vi "DSS-Tests-golden_read.vi"(8 "error in":errorcluster, 11 "file path":path) -> (0 "error out":errorcluster, 2 "found":bool, 3 "values":dbl[](array[numeric]))   [LabVIEW 2020, in "DSS-Tests.lvlib"]
doc: "Reads a golden text file of one value per line (period as decimal point) into a 1D DBL array; found is false and the array empty when the file does not exist."
uses:
  DSS-Tests.lvlib
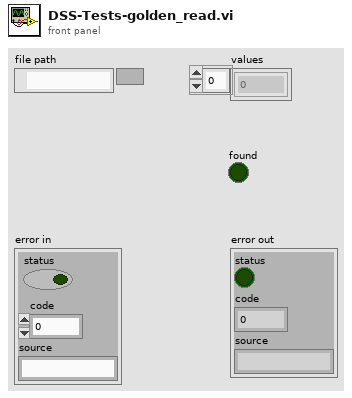
[diagram p1: front panel]
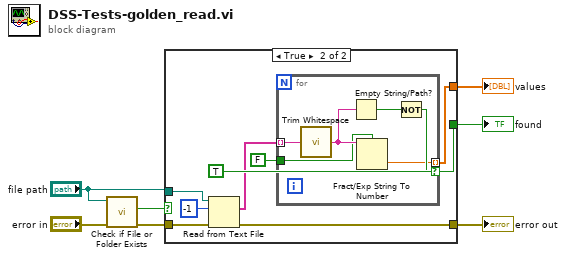
[diagram p0: block diagram]
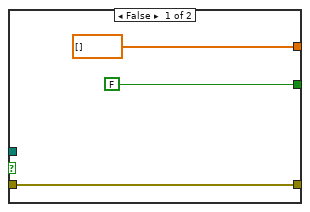
[diagram p2: hidden frame]
diagram:
  n1 = call <vilib>:"Check if File or Folder Exists.vi"("error in (no error)"="error in", "path"="file path") -> ("error out"=w3:errorcluster, "file or folder exists?"=w4:bool)  [unwired: 7 in, 1 out]
  n2 = case shown="True" w4 {
    tunnel: "file path" -> [_ w11]
    tunnel: [FALSE ("not found") TRUE ("found")] -> w6
    tunnel: w3 -> [w8 w12]
    tunnel: [w8 w15] -> w7
    tunnel: [dbl[] [] ("no values") w17] -> w5
    frame False {
    }
    frame True {
      n3 = Read from Text File(file (use dialog)=w11, count=-1, error in=w12) -> (text=w14:string[], error out=w15:errorcluster)  [unwired: 1 in, 2 out]
      n4 = for {
        tunnel: FALSE ("use system decimal point (T)") -> [w20]
        tunnel: w14 -> [w19] mode=indexing
        tunnel: [w22] -> w17 mode=indexing if=w24
        n5 = call <vilib>:"Trim Whitespace.vi"("string"=w19) -> ("trimmed string"=w21:string)  [unwired: 1 in]
        n6 = Empty String/Path?(string/path=w21) -> (empty?=w23:bool)
        n7 = Fract/Exp String To Number(use system decimal point (T)=w20, string=w21) -> (number=w22:dbl)  [unwired: 2 in, 1 out]
        n8 = Not(x=w23) -> (.not. x?=w24:bool)
      }
    }
  }
  "values" <- w5
  "found" <- w6
  "error out" <- w7
